vi "RemoteVI Fixture Find Control.vi"(0 "Panel":refnum<vi>, 5 "label":string, 11 "error in":errorcluster) -> (4 "Control Ref":refnum<vi>, 15 "error out":errorcluster)   [LabVIEW 2020]
doc: "Helper of RemoteVI Fixture.vi. Returns a reference to the top-level control on Panel whose label is label, for registering its events dynamically (the fixture's Tab control is pasted in after generation, so no static event can name it). Not a Refnum when no control carries that label. Errors of the property reads go to error out."
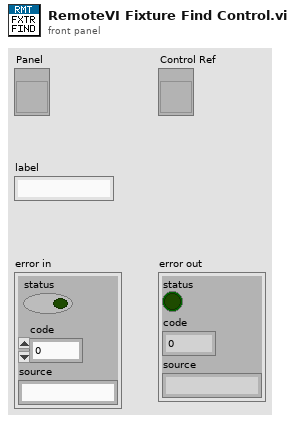
[diagram p1: front panel]
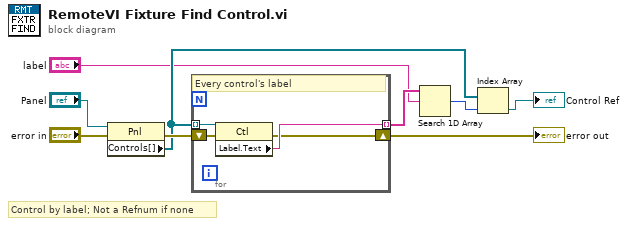
[diagram p0: block diagram]
diagram:
  # "Control by label; Not a Refnum if none"
  n1 = property class="Pnl"(reference="Panel", error in="error in") -> (error out=w5:errorcluster, "Controls[]"=w4:refnum<vi>[])  [unwired: 1 out]
  n2 = for {
    tunnel: w4 -> [w10] mode=indexing
    shift-right: [w12] -> w6
    shift-left: w5 -> [w11]
    tunnel: [w13] -> w7 mode=indexing
    # "Every control's label"
    n3 = property class="Ctl"(reference=w10, error in=w11) -> (error out=w12:errorcluster, "Label.Text"=w13:string)  [unwired: 1 out]
  }
  "error out" <- w6
  n4 = Search 1D Array(1D array=w7, element="label") -> (index of element=w8:i32)  [unwired: 1 in]
  n5 = Index Array(array=w4, index=w8) -> (element=→"Control Ref":refnum<vi>)
